vi "Mock Call.vi"(10 "Control Values":cluster{"Name":string, "Variant Data":variant}[](array[cluster]), 11 "Mock In":refnum<class "LMock Mock.lvclass">) -> (2 "Return Values":map{string, variant}(c390), 3 "Mock Out":refnum<class "LMock Mock.lvclass">)   [LabVIEW 2020, in "LMock Mock.lvclass"]
uses:
  LMock Mock.lvclass
  LMock Mock.lvclass/LMock Mock.ctl
  Parametric VI Call/Parametric VI Call.lvclass
  C:/git/astemes-lmock/source/Core/VI Call/VI Call.lvclass
  Core/VI Call/VI Call.lvclass
  Core/Expectation/Expectation.lvclass
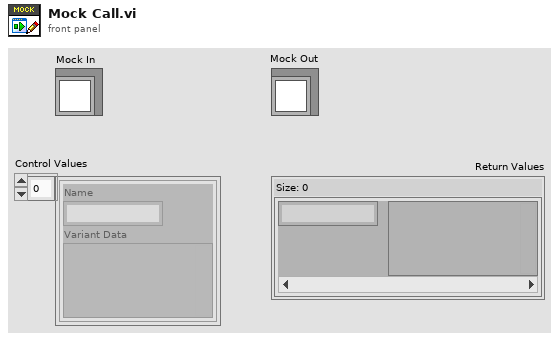
[diagram p1: front panel]
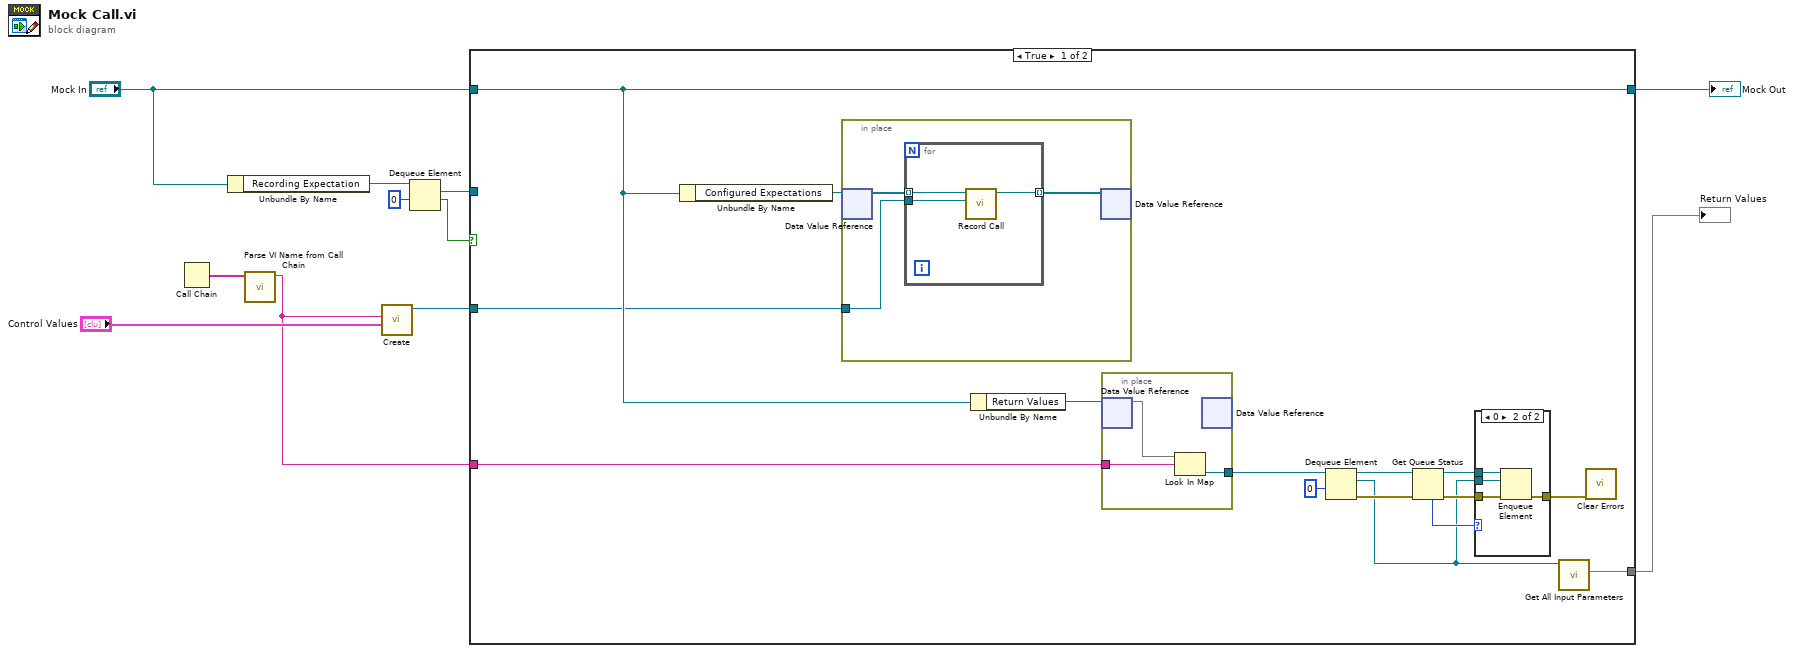
[diagram p0: block diagram]
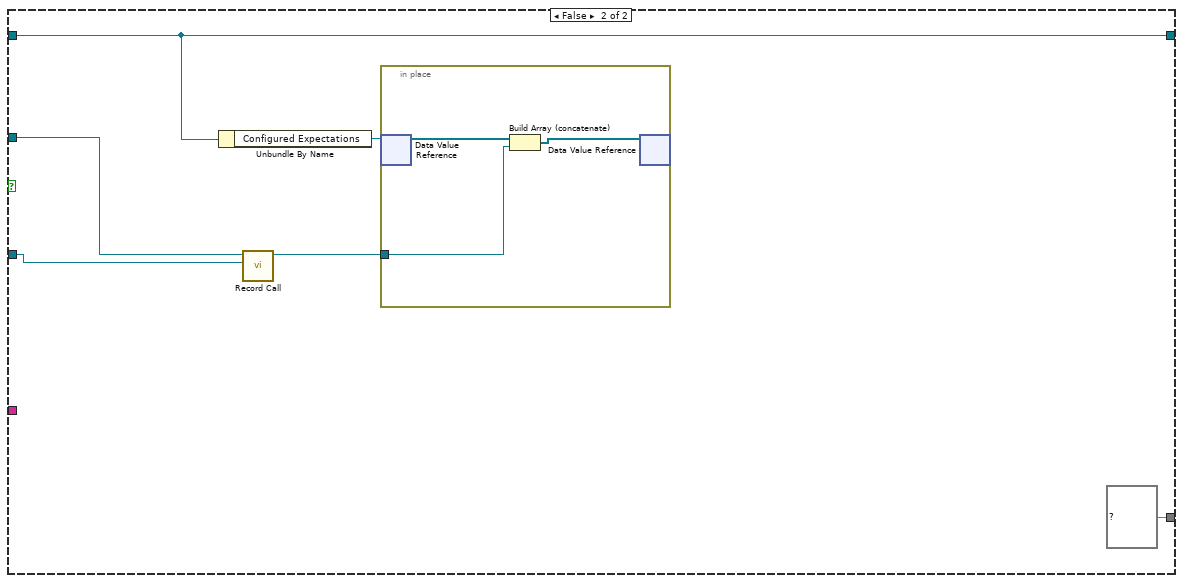
[diagram p3: hidden frame]
diagram:
  n1 = Call Chain() -> (call chain=w5:string[])
  n2 = Unbundle By Name("Mock In") -> ("Recording Expectation"=w9:refnum<queue>)
  n3 = call "Parse VI Name from Call Chain.vi"("call chain"=w5) -> ("VI Name"=w1:string)  [unwired: 10 in]
  n4 = call "Create.vi"("Control Values"="Control Values", "VI Name"=w1) -> ("Parametric VI Call Out"=w3:refnum<class "Parametric VI Call.lvclass">)  [unwired: 9 in]
  n5 = Dequeue Element(queue=w9, timeout in ms (-1)=0) -> (element=w6:refnum<class "Expectation.lvclass">, timed out?=w2:bool)  [unwired: 1 in, 2 out]
  n6 = case shown="True" w2 {
    tunnel: [w15 map{string, variant} {} ("Input Parameters")] -> w11
    tunnel: "Mock In" -> [w14 w45]
    tunnel: [w14 w45] -> w7
    tunnel: w6 -> [_ w43]
    tunnel: w3 -> [w13 w42]
    tunnel: w1 -> [w12 _]
    frame True {
      n7 = Unbundle By Name(w14) -> ("Configured Expectations"=w26:refnum<data-value>)
      n8 = in-place {
        in-place-border: w13 -> [w27]
        n9 = in-place-dvr #1(w26) -> (w29:refnum<class "Expectation.lvclass">[])  [unwired: 1 out]
        n10 = for {
          tunnel: w29 -> [w32] mode=indexing
          tunnel: [w31] -> w28 mode=indexing
          tunnel: w27 -> [w30]
          n11 = call-dynamic "Record Call.vi"("VI Call"=w30, "Expectation in"=w32) -> ("Expectation out"=w31:refnum<class "Expectation.lvclass">)  [unwired: 9 in]
        }
        n12 = in-place-dvr #1(w28) -> ()  [unwired: 2 out]
      }
      n13 = Unbundle By Name(w14) -> ("Return Values"=w25:refnum<data-value>)
      n14 = in-place {
        in-place-border: [w39] -> w24
        in-place-border: w12 -> [w38]
        n15 = in-place-dvr #2(w25) -> (w40:map{string, refnum<queue>})  [unwired: 1 out]
        n16 = Look In Map(map=w40, key=w38) -> (value=w39:refnum<queue>)  [unwired: 1 in, 1 out]
        n17 = in-place-dvr #2() -> ()  [unwired: 1 in, 2 out]
      }
      n18 = Dequeue Element(queue=w24, timeout in ms (-1)=0) -> (queue out=w20:refnum<queue>, element=w16:refnum<class "VI Call.lvclass">, error out=w22:errorcluster)  [unwired: 1 in, 1 out]
      n19 = Get Queue Status(queue=w20, error in (no error)=w22) -> (queue out=w18:refnum<queue>, error out=w21:errorcluster, # elements in queue=w17:i32)  [unwired: 1 in, 5 out]
      n20 = case shown="0" w17 {
        tunnel: w21 -> [w33 w37]
        tunnel: [w33 w36] -> w19
        tunnel: w18 -> [_ w35]
        tunnel: w16 -> [_ w34]
        frame Default {
        }
        frame 0 {
          n21 = Enqueue Element(queue=w35, element=w34, error in (no error)=w37) -> (error out=w36:errorcluster)  [unwired: 1 in, 2 out]
        }
      }
      n22 = call-dynamic "Get All Input Parameters.vi"("VI Call in"=w16) -> ("Input Parameters"=w15:map{string, variant})  [unwired: 9 in, 1 out]
      n23 = call <vilib>:"Clear Errors.vi"("error in (no error)"=w19) -> ()  [unwired: 5 in, 2 out]
    }
    frame False {
      n24 = Unbundle By Name(w45) -> ("Configured Expectations"=w46:refnum<data-value>)
      n25 = call-dynamic "Record Call.vi"("VI Call"=w42, "Expectation in"=w43) -> ("Expectation out"=w41:refnum<class "Expectation.lvclass">)  [unwired: 9 in]
      n26 = in-place {
        in-place-border: w41 -> [w47]
        n27 = in-place-dvr #3(w46) -> (w49:refnum<class "Expectation.lvclass">[])  [unwired: 1 out]
        n28 = Build Array (concatenate)(w49, w47) -> (w48:refnum<class "Expectation.lvclass">[])
        n29 = in-place-dvr #3(w48) -> ()  [unwired: 2 out]
      }
    }
  }
  "Mock Out" <- w7
  "Return Values" <- w11
